vi "Log.vi"(8 "error in":errorcluster, 10 "Log Entry":T1 {"Time" format="%<%x %.3X>T"}, 11 "File Logger in":refnum<class "File Logger.lvclass">) -> (0 "error out":errorcluster, 3 "File Logger out":refnum<class "File Logger.lvclass">)   [LabVIEW 2026, in "File Logger.lvlib" / "File Logger.lvclass"]
doc: "Log the provided entry."
uses:
  File Logger.lvclass
  Type Definitions/Log Entry--cluster.ctl
  File Logger.lvclass/File Logger.ctl
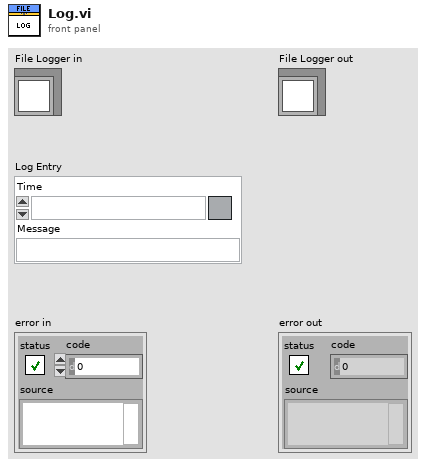
[diagram p1: front panel]
types:
  T1 = typedef "Log Entry--cluster.ctl" = cluster{"Time":timestamp, "Message":string}
  T2 = enum16{"open", "replace", "create", "open or create", "replace or create", "replace or create with confirmation"}
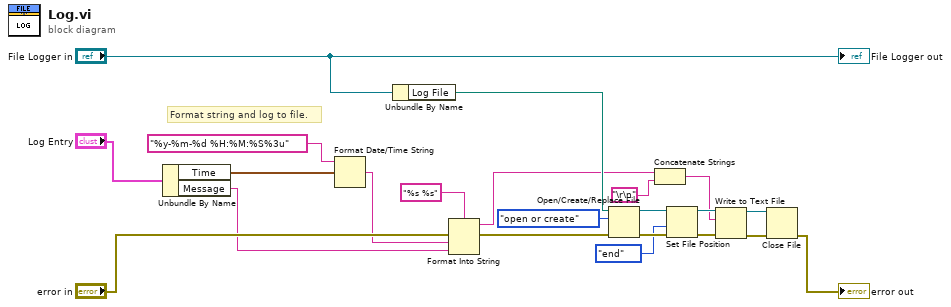
[diagram p0: block diagram]
diagram:
  # "Format string and log to file."
  n1 = Unbundle By Name("Log Entry") -> ("Time"=w16:timestamp, "Message"=w12:string)
  n2 = Format Date/Time String(time format string (%c)="%y-%m-%d %H:%M:%S%3u", seconds (now)=w16) -> (date/time string=w13:string)  [unwired: 1 in]
  n3 = Unbundle By Name("File Logger in") -> ("Log File"=w7:path)
  n4 = Format Into String(format string="%s %s", error in="error in", w13, w12) -> (resulting string=w2:string, error out=w20:errorcluster)  [unwired: 1 in]
  n5 = Open/Create/Replace File(file path (use dialog)=w7, error in=w20, operation (0:open)=T2."open or create") -> (refnum out=w9:refnum<file>, error out=w21:errorcluster)  [unwired: 3 in, 1 out]
  n6 = Concatenate Strings(w2, "\r\n") -> (w4:string)
  n7 = Set File Position(refnum=w9, from (0:start)=enum16{"start", "end", "current"}."end", error in=w21) -> (refnum out=w5:refnum<file>, error out=w19:errorcluster)  [unwired: 1 in]
  n8 = Write to Text File(file (use dialog)=w5, text=w4, error in=w19) -> (refnum out=w3:refnum<file>, error out=w18:errorcluster)  [unwired: 1 in, 1 out]
  n9 = Close File(refnum=w3, error in=w18) -> (error out=→"error out":errorcluster)  [unwired: 1 out]
  "File Logger out" <- "File Logger in"
